vi "get channel buffer from batch buffer.vi"(9 "channel tags":cluster{"key":string, "value":string}[](array[cluster]), 10 "channel":string, 11 "batch buffer":refnum<data-value>) -> (0 "error out":errorcluster, 3 "channel point buffer":refnum<data-value>)   [LabVIEW 2020, in "nominal core steps.lvlib"]
doc: "In the batch buffer, register a channel by name and tag and get a direct reference to the underlying buffer, or look up an existing buffer. \n\nTags are part of the unique identification of a channel, but are not required.\n\nExamples:\nCall with \"name\", <no tags>; Call with \"name\", <no tags> => one channel\nCall with \"name\", <no tags>; Call with \"name\", tags: [sn: 123] => two channels\nCall with \"name\", tags: [sn: 123]; Call with \"name\", tags: [sn: 321] => two channels"
uses:
  nominal core steps.lvlib
  batch buffer.ctl
  channel uid.ctl
  points buffer.ctl
  single point.ctl
  <vilib>/Utility/miscctls.llb/LVMapReplaceAction.ctl
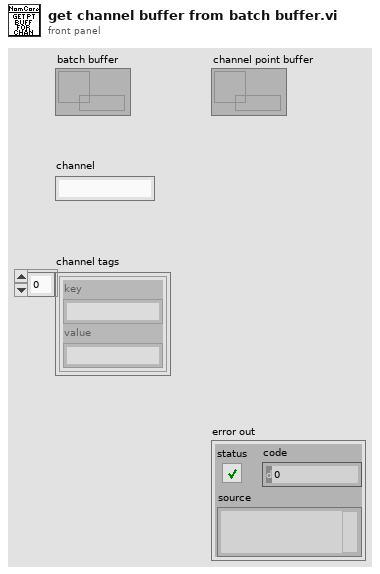
[diagram p1: front panel]
types:
  T1 = typedef "nominal core steps.lvlib/channel uid.ctl" = cluster{"channel name":string, "tags":map{string, string}}
  T2 = typedef "LVMapReplaceAction.ctl" = enum32{"Modify Entry only if found", "Add or Modify Entry", "Delete Entry"}
  T3 = typedef "nominal core steps.lvlib/batch buffer.ctl" = map{T1, refnum<data-value>}
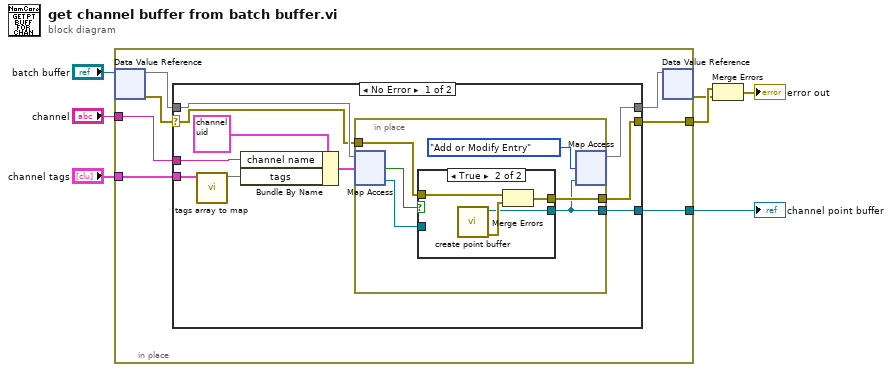
[diagram p0: block diagram]
diagram:
  n1 = in-place {
    in-place-border: [w13] -> w6
    in-place-border: "channel" -> [w10]
    in-place-border: "channel tags" -> [w9]
    in-place-border: [w8] -> w1
    n2 = in-place-dvr #1("batch buffer") -> (w12:T3, w14:errorcluster)
    n3 = case shown="No Error" w14 {
      selector: w14 -> [w22 w38]
      tunnel: [w16 w38] -> w13
      tunnel: w12 -> [w24 w37]
      tunnel: [w23 w37] -> w11
      tunnel: w10 -> [w19 _]
      tunnel: w9 -> [w21 _]
      tunnel: [w15 _] -> w8
      frame No Error {
        n4 = call "tags array to map.vi"("channel tags"=w21) -> ("map"=w18:map{string, string})  [unwired: 10 in]
        n5 = Bundle By Name(cluster=T1 {"channel name"="", "tags"={}} ("channel unique identifier"), "channel name"=w19, "tags"=w18) -> (w17:T1)
        n6 = in-place {
          in-place-border: w22 -> [w27]
          in-place-border: [w26] -> w16
          in-place-border: [w25] -> w15
          n7 = in-place-map #2(w24, w17) -> (w29:refnum<data-value>, w28:bool)  [unwired: 1 in]
          n8 = case shown="True" w28 {
            tunnel: w29 -> [w31 _]
            tunnel: w27 -> [w32 w36]
            tunnel: [w32 w34] -> w26
            tunnel: [w31 w33] -> w25
            frame False {
            }
            frame True {
              n9 = call "create point buffer.vi"() -> ("error out"=w35:errorcluster, "point buffer"=w33:refnum<data-value>)  [unwired: 10 in]
              n10 = Merge Errors(w36, w35) -> (w34:errorcluster)
            }
          }
          n11 = in-place-map #2(w25, LVMapReplaceAction."Add or Modify Entry" ("action")) -> (w23:T3)  [unwired: 2 out]
        }
      }
      frame Error {
      }
    }
    n12 = in-place-dvr #1(w11) -> (w5:errorcluster)  [unwired: 1 out]
  }
  "channel point buffer" <- w1
  n13 = Merge Errors(w6, w5) -> (→"error out":errorcluster)
